vi "Start Sync.vi"(8 "error in (no error)":errorcluster, 11 "gRPC Server in":refnum<class "GreeterService.lvclass">) -> (0 "error out":errorcluster, 3 "gRPC Server out":refnum<class "GreeterService.lvclass">)   [LabVIEW 2019, in "Generated_server.lvlib" / "GreeterService.lvclass"]
uses:
  GreeterService.lvclass
  GreeterService.lvclass/GreeterService.ctl
  RPC Messages/Greeter_res.ctl
  RPC Messages/Greeter_res_res_oneof/Greeter_res_res_oneof.lvclass
  RPC Messages/Greeter_req_req_oneof/Greeter_req_req_oneof.lvclass/Greeter_req_req_oneof.ctl
  RPC Messages/Greeter_MessageA.ctl
  RPC Messages/Greeter_MessageA_oneof_a/Greeter_MessageA_oneof_a.lvclass
  RPC Messages/Greeter_MessageA_oneof_a/Greeter_MessageA_oneof_a.lvclass/Greeter_MessageA_oneof_a.ctl
  RPC Messages/Greeter_res_res_oneof/Greeter_res_res_oneof.lvclass/Greeter_res_res_oneof.ctl
  Generated_server.lvlib
  RPC Messages/Greeter_req_req_oneof/Greeter_req_req_oneof.lvclass
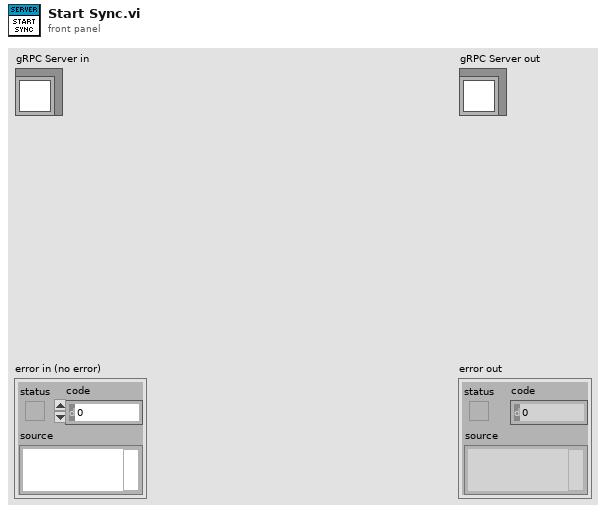
[diagram p1: front panel]
types:
  T1 = typedef "Generated_server.lvlib/Greeter_res.ctl" = cluster{"res_id":i32, "Greeter_res_res_oneof":refnum<class "Greeter_res_res_oneof.lvclass">}
  T2 = typedef "Generated_server.lvlib/Greeter_MessageA.ctl" = cluster{"anotherField":string, "Greeter_MessageA_oneof_a":refnum<class "Greeter_MessageA_oneof_a.lvclass">}
  T3 = typedef "Generated_server.lvlib/GreeterService.lvclass/Server Internal UEs.ctl" = cluster{"GreeterService GetFeature Internal UE":refnum<user-event>}
  T4 = typedef "Generated_server.lvlib/GreeterService.lvclass/Server gRPC UEs.ctl" = cluster{"GreeterService GetFeature gRPC UE":refnum<user-event>}
  T5 = typedef "grpc-lvsupport-release.lvlib/grpcId.ctl" = u64
  T6 = typedef "Generated_server.lvlib/Greeter_req.ctl" = cluster{"req_id":i32, "Greeter_req_req_oneof":refnum<class "Greeter_req_req_oneof.lvclass">}
  T7 = typedef "grpc-lvsupport.lvlib/grpcId.ctl" = u64
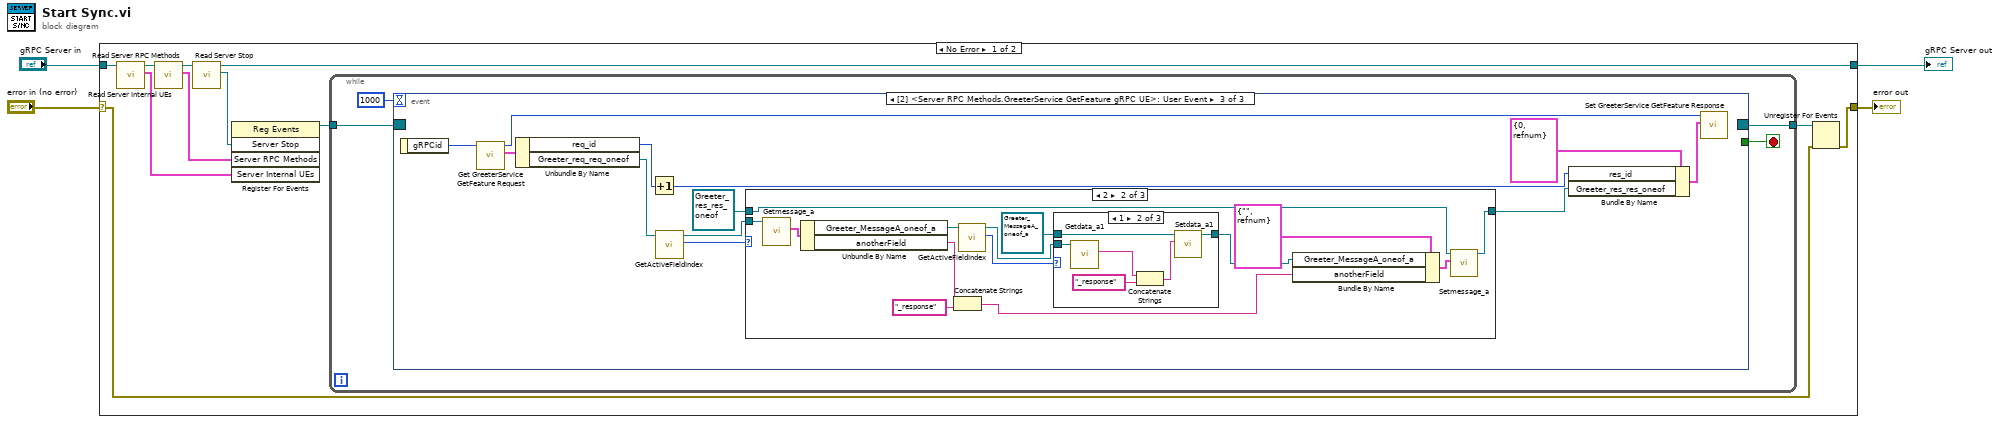
[diagram p0: block diagram]
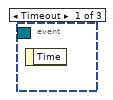
[diagram p2: hidden frame]
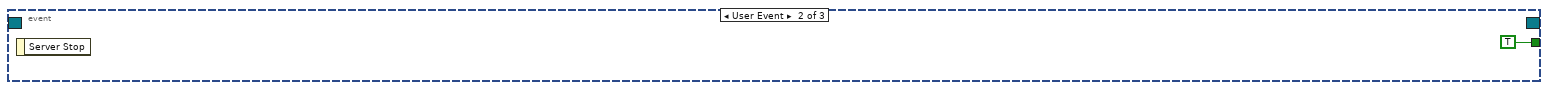
[diagram p3: hidden frame]
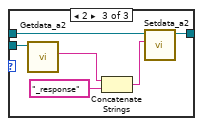
[diagram p6: hidden frame]
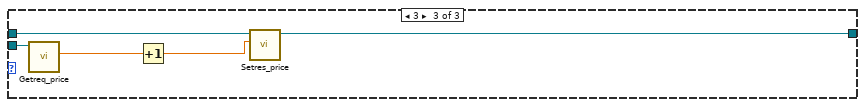
[diagram p7: hidden frame]
diagram:
  n1 = case shown="No Error" "error in (no error)" {
    selector: "error in (no error)" -> [w9 w67]
    tunnel: [w8 w67] -> w3
    tunnel: [w6 w66] -> w1
    tunnel: "gRPC Server in" -> [w15 w66]
    frame No Error {
      n2 = call "Read Server Internal UEs.vi"("SignalGeneratorService in"=w15) -> ("Server Internal UEs"=w13:T3, "SignalGeneratorService out"=w14:refnum<class "GreeterService.lvclass">)  [unwired: 8 in, 1 out]
      n3 = call "Read Server RPC Methods.vi"("SignalGeneratorService in"=w14) -> ("Server RPC Methods"=w7:T4, "SignalGeneratorService out"=w12:refnum<class "GreeterService.lvclass">)  [unwired: 8 in, 1 out]
      n4 = call-dynamic "Read Server Stop.vi"("iService in"=w12) -> ("Server Stop"=w5:refnum<user-event>, "iService out"=w6:refnum<class "GreeterService.lvclass">)  [unwired: 8 in, 1 out]
      n5 = register-events(w5, w7, w13) -> (reference out=w11:refnum<event-registration>)  [unwired: 2 in, 1 out]
      n6 = while {
        tunnel: w11 -> [w19]
        tunnel: [w17] -> w10
        stop <- w18 stop-if-true
        n7 = event "RPC Methods Event Structure" shown="[2] <Server RPC Methods.GreeterService GetFeature gRPC UE>: User Event" {
          selector: w19 -> [_ _ _]
          dyn-events: [_ _ _] -> w17
          timeout: 1000 -> [_ _ _]
          tunnel: [_ TRUE _] -> w18
          event Timeout {
            n8 = event-data() -> ()  [unwired: 1 in, 1 out]
          }
          event User Event {
            n9 = event-data() -> ()  [unwired: 1 in, 1 out]
          }
          event User Event {
            n10 = event-data() -> ("gRPCid"=w32:T5)  [unwired: 1 in]
            n11 = call "Get GreeterService GetFeature Request.vi"("gRPCid in"=w32) -> ("Message Data"=w31:T6, "gRPCid out"=w27:T7)  [unwired: 8 in, 1 out]
            n12 = Unbundle By Name(w31) -> ("req_id"=w25:i32, "Greeter_req_req_oneof"=w29:refnum<class "Greeter_req_req_oneof.lvclass">)
            n13 = Increment(x=w25) -> (x+1=w21:i32)
            n14 = call "GetActiveFieldIndex.vi"("OneOfTemplate in"=w29) -> ("Active Field Index"=w26:i32, "OneOfTemplate out"=w28:refnum<class "Greeter_req_req_oneof.lvclass">)  [unwired: 8 in, 1 out]
            n15 = case shown="2" w26 {
              tunnel: w28 -> [_ w43 w65]
              tunnel: [w33 w42 w61] -> w23
              tunnel: refnum<class "Greeter_res_res_oneof.lvclass"> refnum ("OneOfTemplate in") -> [w33 w41 w62]
              frame 0, Default {
              }
              frame 2 {
                n16 = call "Getmessage_a.vi"("OneOfTemplate in"=w43) -> ("Get_Val"=w47:T2)  [unwired: 8 in, 2 out]
                n17 = Unbundle By Name(w47) -> ("Greeter_MessageA_oneof_a"=w46:refnum<class "Greeter_MessageA_oneof_a.lvclass">, "anotherField"=w36:string)
                n18 = Concatenate Strings(w36, "_response" ("string")) -> (w35:string)
                n19 = call "GetActiveFieldIndex.vi"("OneOfTemplate in"=w46) -> ("Active Field Index"=w45:i32, "OneOfTemplate out"=w44:refnum<class "Greeter_MessageA_oneof_a.lvclass">)  [unwired: 8 in, 1 out]
                n20 = case shown="1" w45 {
                  tunnel: w44 -> [_ w54 w59]
                  tunnel: refnum<class "Greeter_MessageA_oneof_a.lvclass"> refnum ("OneOfTemplate in") -> [w48 w50 w56]
                  tunnel: [w48 w49 w55] -> w39
                  frame 0, Default {
                  }
                  frame 1 {
                    n21 = call "Getdata_a1.vi"("OneOfTemplate in"=w54) -> ("Get_Val"=w53:string)  [unwired: 8 in, 2 out]
                    n22 = Concatenate Strings(w53, "_response" ("string")) -> (w51:string)
                    n23 = call "Setdata_a1.vi"("Set_Val"=w51, "OneOfTemplate in"=w50) -> ("OneOfTemplate out"=w49:refnum<class "Greeter_MessageA_oneof_a.lvclass">)  [unwired: 8 in, 1 out]
                  }
                  frame 2 {
                    n24 = call "Getdata_a2.vi"("OneOfTemplate in"=w59) -> ("Get_Val"=w58:string)  [unwired: 8 in, 2 out]
                    n25 = Concatenate Strings(w58, "_response" ("string")) -> (w57:string)
                    n26 = call "Setdata_a2.vi"("Set_Val"=w57, "OneOfTemplate in"=w56) -> ("OneOfTemplate out"=w55:refnum<class "Greeter_MessageA_oneof_a.lvclass">)  [unwired: 8 in, 1 out]
                  }
                }
                n27 = Bundle By Name(cluster=T2 {"anotherField"="", "Greeter_MessageA_oneof_a"=refnum} ("Greeter_MessageA"), "Greeter_MessageA_oneof_a"=w39, "anotherField"=w35) -> (w37:T2)
                n28 = call "Setmessage_a.vi"("Set_Val"=w37, "OneOfTemplate in"=w41) -> ("OneOfTemplate out"=w42:refnum<class "Greeter_res_res_oneof.lvclass">)  [unwired: 8 in, 1 out]
              }
              frame 3 {
                n29 = call "Getreq_price.vi"("OneOfTemplate in"=w65) -> ("Get_Val"=w64:dbl)  [unwired: 8 in, 2 out]
                n30 = Increment(x=w64) -> (x+1=w63:dbl)
                n31 = call "Setres_price.vi"("Set_Val"=w63, "OneOfTemplate in"=w62) -> ("OneOfTemplate out"=w61:refnum<class "Greeter_res_res_oneof.lvclass">)  [unwired: 8 in, 1 out]
              }
            }
            n32 = Bundle By Name(cluster=T1 {"res_id"=0, "Greeter_res_res_oneof"=refnum} ("Greeter_res"), "res_id"=w21, "Greeter_res_res_oneof"=w23) -> (w24:T1)
            n33 = call "Set GreeterService GetFeature Response.vi"("Message Data"=w24, "gRPCid in"=w27) -> ()  [unwired: 9 in, 1 out]
          }
        }
      }
      n34 = Unregister For Events(event registration refnum=w10, error in=w9) -> (error out=w8:errorcluster)
    }
    frame Error {
    }
  }
  "error out" <- w3
  "gRPC Server out" <- w1
